vi "WS_Handshake.vi"(8 "error in (no error)":errorcluster, 9 "channel":u8, 10 "host":string, 11 "TLS connection":refnum<k5>) -> (0 "error out":errorcluster, 1 "headers":string, 2 "leftover":u8[](array[numeric]), 3 "TLS connection out":refnum<k5>)   [LabVIEW 2021, in "CANsub_Common.lvlib"]
doc: "Sends the WebSocket upgrade for /api/can/<channel>/ws on an open TLS connection and reads the reply headers (max 2 s). Error 5004 if the status is not 101. Bytes after the headers come out as leftover; feed them to the decoder before the first TCP Read. Uses the RFC 6455 example key; Sec-WebSocket-Accept is not checked."
uses:
  CANsub_Common.lvlib
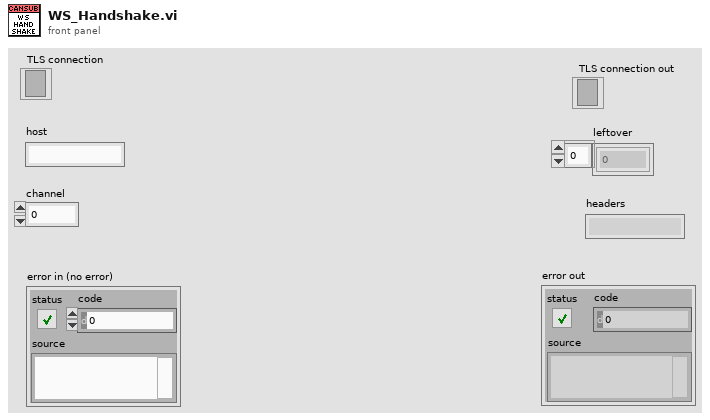
[diagram p1: front panel]
types:
  T1 = enum16{"Standard", "Buffered", "CRLF", "Immediate"}
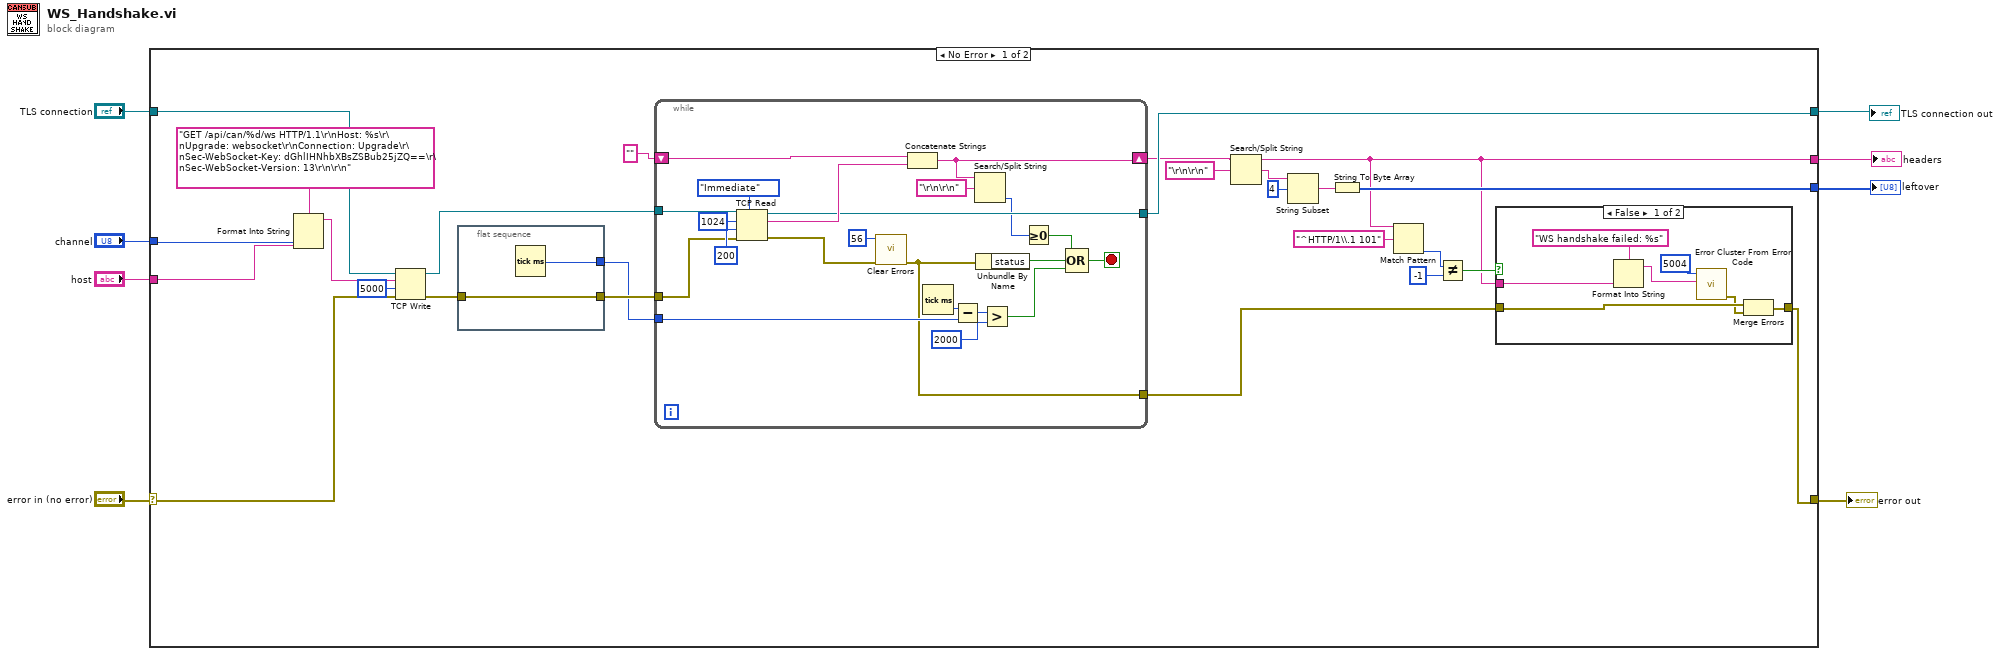
[diagram p0: block diagram]
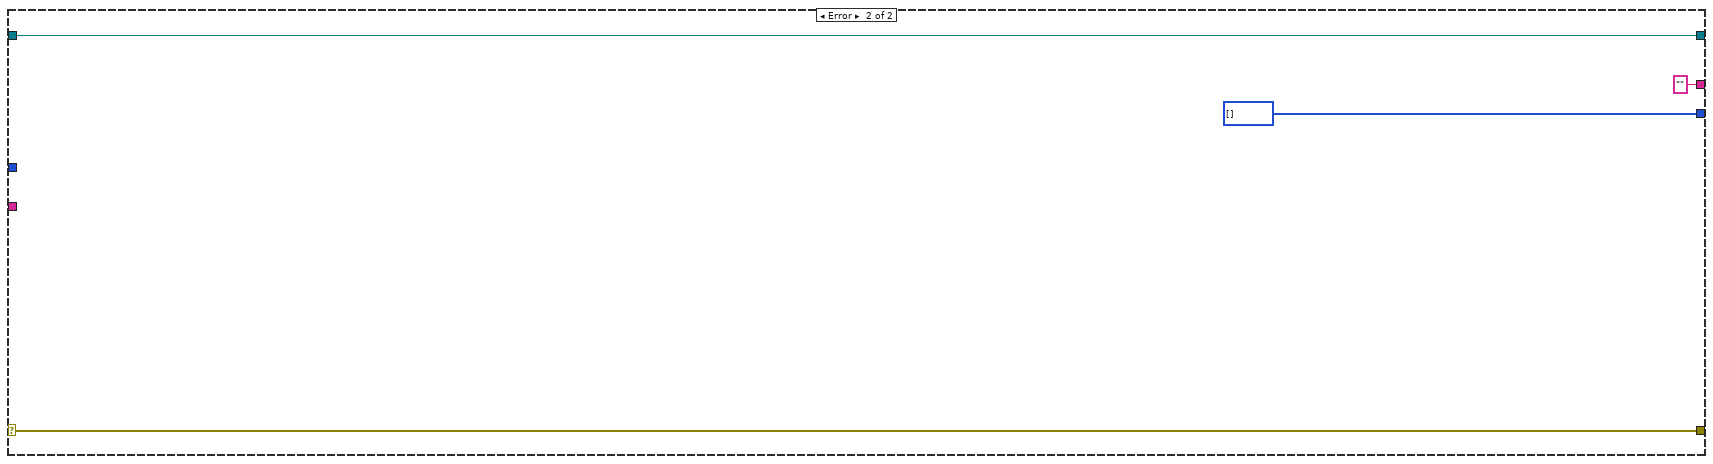
[diagram p3: hidden frame]
diagram:
  n1 = case shown="No Error" "error in (no error)" {
    selector: "error in (no error)" -> [w27 w70]
    tunnel: "channel" -> [w33 _]
    tunnel: "host" -> [w32 _]
    tunnel: "TLS connection" -> [w31 w69]
    tunnel: [w10 w70] -> w4
    tunnel: [w23 w69] -> w3
    tunnel: [w9 ""] -> w2
    tunnel: [w16 u8[] [] ("unsigned byte array")] -> w1
    frame No Error {
      n2 = Format Into String(format string="GET /api/can/%d/ws HTTP/1.1\r\nHost: %s\r\nUpgrade: websocket\r\nConnection: Upgrade\r\nSec-WebSocket-Key: dGhlIHNhbXBsZSBub25jZQ==\r\nSec-WebSocket-Version: 13\r\n\r\n", w33, w32) -> (resulting string=w30:string)  [unwired: 2 in, 1 out]
      n3 = TCP Write(connection ID=w31, data in=w30, error in (no error)=w27, 9:5000 ("timeout ms (25000)")) -> (connection ID out=w25:refnum<k5>, error out=w28:errorcluster)  [unwired: 1 out]
      n4 = flat-sequence {
        tunnel: [w66] -> w22
        tunnel: [w65] -> w24
        tunnel: w28 -> [w65]
        frame #0 {
          n5 = Tick Count (ms)() -> (millisecond timer value=w66:u32)
        }
      }
      n6 = while {
        shift-right: [w54] -> w20
        shift-left: "" -> [w59]
        tunnel: w25 -> [w62]
        tunnel: w24 -> [w60]
        tunnel: [w55] -> w23
        tunnel: w22 -> [w50]
        tunnel: [w43] -> w11
        stop <- w44 stop-if-true
        n7 = TCP Read(connection ID=w62, bytes to read=1024, error in (no error)=w60, 7:T1."Immediate" ("mode (standard)"), 9:200 ("timeout ms (25000)")) -> (connection ID out=w55:refnum<k5>, data out=w58:string, error out=w57:errorcluster)
        n8 = call <vilib>:"Clear Errors.vi"("error in (no error)"=w57, "specific error code to clear (0: all)"=56) -> ("error out"=w43:errorcluster)  [unwired: 4 in, 1 out]
        n9 = Concatenate Strings(w59, w58) -> (w54:string)
        n10 = Tick Count (ms)() -> (millisecond timer value=w51:u32)
        n11 = Subtract(x=w51, y=w50) -> (x-y=w49:u32)
        n12 = Search/Split String(string=w54, search string/char (-)="\r\n\r\n") -> (offset of match=w52:i32)  [unwired: 1 in, 2 out]
        n13 = Unbundle By Name(w43) -> ("status"=w46:bool)
        n14 = Greater?(x=w49, y=u32 2000) -> (0:w45:bool)
        n15 = Greater Or Equal To 0?(x=w52) -> (x >= 0?=w47:bool)
        n16 = Compound Arithmetic op=OR(w47, w46, w45) -> (w44:bool)
      }
      n17 = Search/Split String(string=w20, search string/char (-)="\r\n\r\n") -> (substring before match=w9:string, match + rest of string=w19:string)  [unwired: 1 in, 1 out]
      n18 = String Subset(string=w19, offset (0)=4) -> (substring=w17:string)  [unwired: 1 in]
      n19 = String To Byte Array(string=w17) -> (unsigned byte array=w16:u8[])
      n20 = Match Pattern(string=w9, regular expression="^HTTP/1\\.1 101") -> (offset past match=w14:i32)  [unwired: 1 in, 3 out]
      n21 = Not Equal?(x=w14, y=-1) -> (x != y?=w12:bool)
      n22 = case shown="False" w12 {
        tunnel: [w37 w42] -> w10
        tunnel: w11 -> [w36 w42]
        tunnel: w9 -> [w40 _]
        frame False {
          n23 = Format Into String(format string="WS handshake failed: %s", w40) -> (resulting string=w38:string)  [unwired: 2 in, 1 out]
          n24 = call <vilib>:"Error Cluster From Error Code.vi"("error message (\"\")"=w38, "error code (0)"=5004) -> ("error out"=w35:errorcluster)  [unwired: 7 in]
          n25 = Merge Errors(w36, w35) -> (w37:errorcluster)
        }
        frame True {
        }
      }
    }
    frame Error {
    }
  }
  "error out" <- w4
  "TLS connection out" <- w3
  "leftover" <- w1
  "headers" <- w2
